vi "Save User Devices.vi"(8 "error in (no error)":errorcluster, 11 "picoG in":refnum<class "picoG.lvclass">) -> (0 "error out":errorcluster, 3 "picoG out":refnum<class "picoG.lvclass">)   [LabVIEW 2020, in "PicoG-App.lvlib" / "picoG.lvclass"]
uses:
  picoG.lvclass
  picoG.lvclass/picoG.ctl
  <vilib>/Utility/config.llb/Write Key (I32).vi
  PicoG-App.lvlib
  <vilib>/Utility/config.llb/NI_LVConfig.lvlib
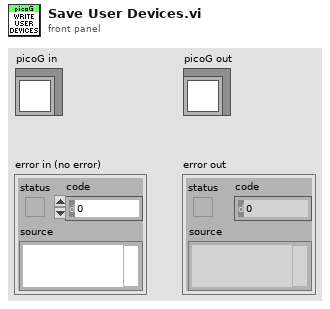
[diagram p1: front panel]
types:
  T1 = typedef "PicoG-App.lvlib/Paths.ctl" = cluster{"User picoG":path, "System picoG":path, "User Config":path, "System Config":path}
  T2 = typedef "NI_LVConfig.lvlib/Config Data RefNum.ctl" = refnum<k1>
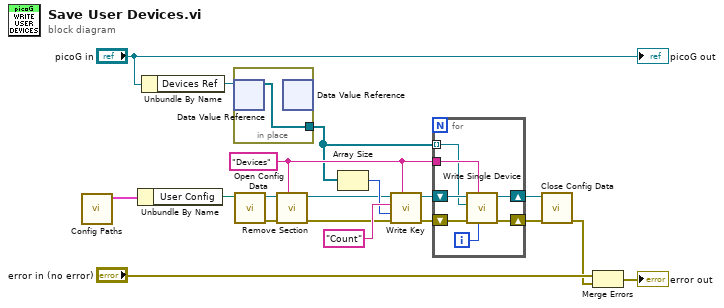
[diagram p0: block diagram]
diagram:
  w4 = "Devices" ("section")
  n1 = call "Config Paths.vi"() -> ("Paths"=w18:T1)  [unwired: 8 in, 3 out]
  n2 = Unbundle By Name(w18) -> ("User Config"=w17:path)
  n3 = Unbundle By Name("picoG in") -> ("Devices Ref"=w3:refnum<data-value>)
  n4 = in-place {
    in-place-border: [w20] -> w1
    n5 = in-place-dvr #1(w3) -> (w20:refnum<class "Device.lvclass">[])  [unwired: 1 out]
    n6 = in-place-dvr #1() -> ()  [unwired: 1 in, 2 out]
  }
  n7 = call <vilib>:"Open Config Data.vi"("configuration file path"=w17) -> ("error out"=w15:errorcluster, "refnum"=w16:T2)  [unwired: 8 in, 1 out]
  n8 = call <vilib>:"Remove Section.vi"("section"=w4, "error in (no error)"=w15, "refnum"=w16) -> ("error out"=w12:errorcluster, "refnum out"=w11:T2)  [unwired: 6 in, 1 out]
  n9 = Array Size(array=w1) -> (size(s)=w13:i32)
  n10 = call-poly <vilib>:"Write Key.vi"("section"=w4, "error in (no error)"=w12, "value"=w13, "key"="Count", "refnum"=w11) -> ("error out"=w10:errorcluster, "refnum out"=w9:T2)  [unwired: 4 in, 1 out]
  n11 = for {
    shift-right: [w22] -> w7
    shift-left: w10 -> [w26]
    shift-right: [w21] -> w8
    shift-left: w9 -> [w27]
    tunnel: w4 -> [w25]
    tunnel: w1 -> [w24] mode=indexing
    i -> [w23]
    n12 = call "Write Single Device.vi"("Index"=w23, "Section"=w25, "error in (no error)"=w26, "Device"=w24, "refnum"=w27) -> ("error out"=w22:errorcluster, "refnum out"=w21:T2)  [unwired: 5 in]
  }
  n13 = call <vilib>:"Close Config Data.vi"("error in (no error)"=w7, "refnum"=w8) -> ("error out"=w5:errorcluster)  [unwired: 8 in, 1 out]
  n14 = Merge Errors("error in (no error)", w5) -> (→"error out":errorcluster)
  "picoG out" <- "picoG in"
